vi "VIH UI - Test Path.vi"(8 "Ena Empty (F)":bool, 9 "Folder (F)":bool, 11 "Path":path) -> (0 "Symbol":i32, 1 "Color":u32(colorbox), 2 "Good Path":bool, 3 "dup Path":path)   [LabVIEW 2014]
doc: "::: VI Helpeks :::\nCopyright (c) 2000-2026 Konstantin Shifershteyn. All rights reserved."
panel:
  # "VI Helpeks\nCopyright (c) 2012-2026 Konstantin Shifershteyn"
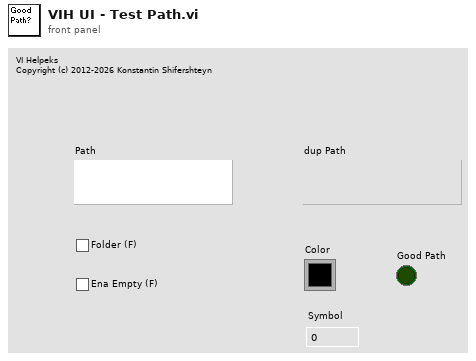
[diagram p1: front panel]
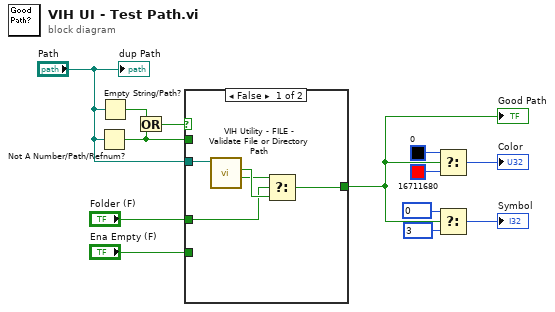
[diagram p0: block diagram]
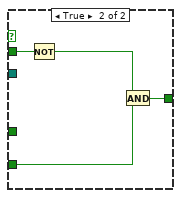
[diagram p2: hidden frame]
diagram:
  n1 = Not A Number/Path/Refnum?(number/path/refnum="Path") -> (NaN/Path/Refnum?=w5:bool)
  n2 = Empty String/Path?(string/path="Path") -> (empty?=w12:bool)
  n3 = Or(x=w12, y=w5) -> (x .or. y?=w11:bool)
  n4 = case shown="False" w11 {
    tunnel: "Path" -> [w18 _]
    tunnel: "Folder (F)" -> [w15 _]
    tunnel: [w14 w21] -> w1
    tunnel: w5 -> [_ w22]
    tunnel: "Ena Empty (F)" -> [_ w19]
    frame False {
      n5 = call "VIH Utility - FILE - Validate File or Directory Path.vi"("Path"=w18) -> ("directory"=w16:bool, "file"=w17:bool)  [unwired: 6 in, 3 out]
      n6 = Select(t=w16, s=w15, f=w17) -> (s? t:f=w14:bool)
    }
    frame True {
      n7 = Not(x=w22) -> (.not. x?=w20:bool)
      n8 = And(x=w20, y=w19) -> (x .and. y?=w21:bool)
    }
  }
  "Good Path" <- w1
  n9 = Select(t=u32 0, s=w1, f=u32 16711680) -> (s? t:f=→"Color":u32)
  n10 = Select(t=0, s=w1, f=3) -> (s? t:f=→"Symbol":i32)
  "dup Path" <- "Path"
